vi "Progress Bar Front Panel.vi"(7 "Enable Cancel?":bool, 8 "Calling VI Ref":refnum<vi>, 9 "Main Title":string, 10 "Progress Bar Dialog":refnum<class "Loading Dialog.lvclass">, 11 "Total":i32) -> ()   [LabVIEW 2020, in "VI Properties Editor.lvlib" / "Loading Dialog.lvclass"]
doc: "The front panel for the dialog box that gets displayed."
uses:
  Loading Dialog.lvclass
  Loading Dialog.lvclass/Loading Dialog.ctl
  VI Properties Editor.lvlib
panel:
  in  "Cancelling":string="Cancelling..."
  in  "Progress Format String":string="%d of %s"
  out "Main Heading":string="Loading item data..."
  in  "Cancel":bool
  out "Status Heading":string="0 of 0"
  out "Progress Bar":dbl(slide) scale=0.0..1.0
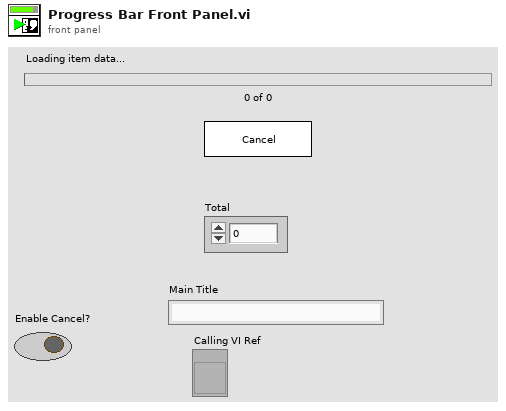
[diagram p1: front panel]
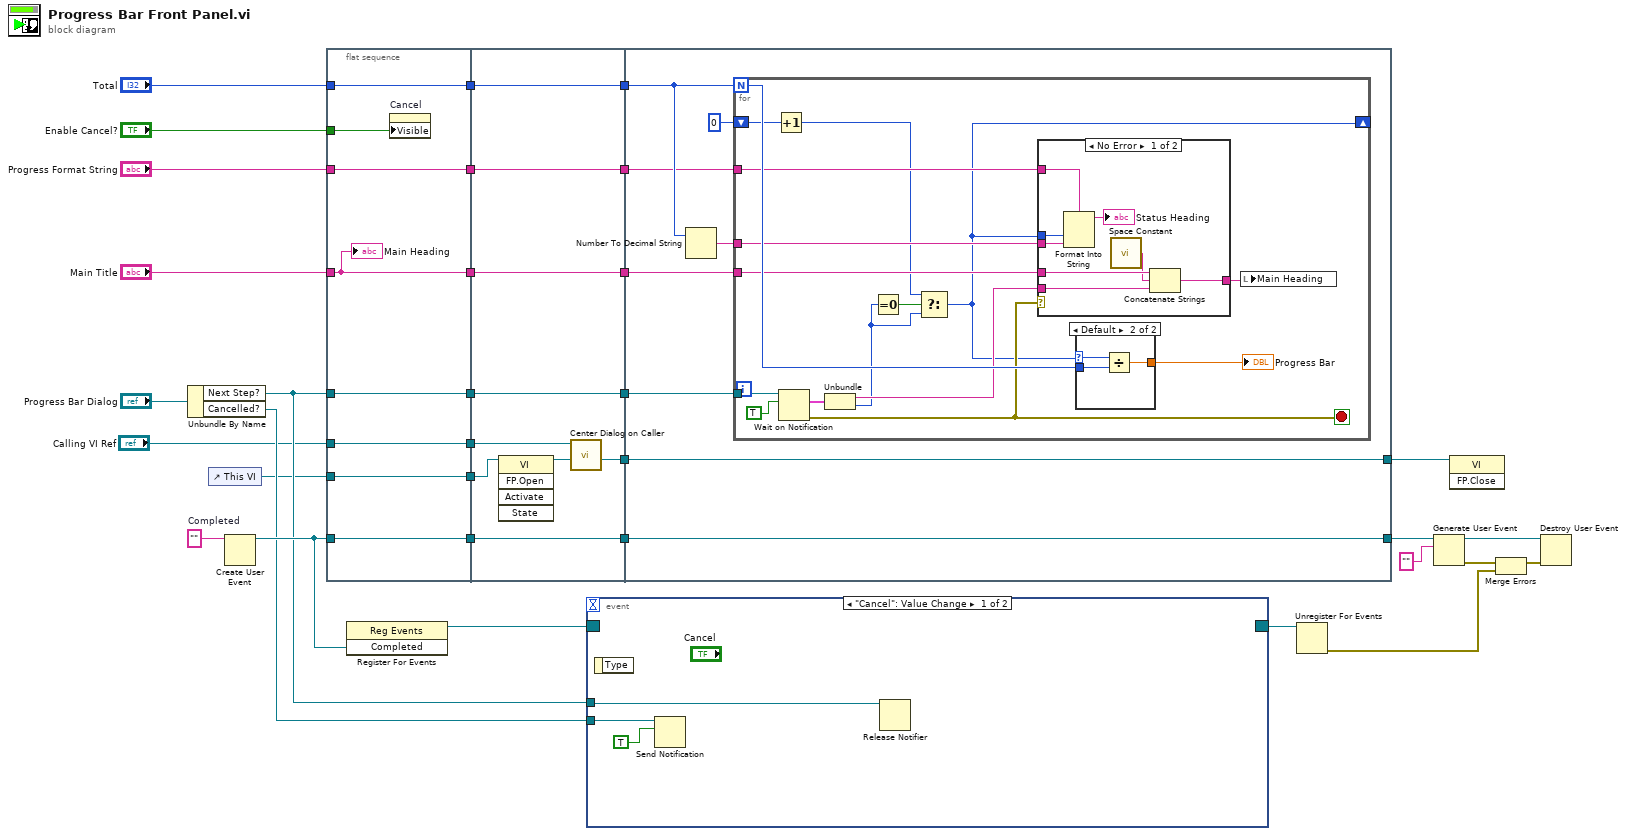
[diagram p0: block diagram]
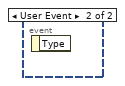
[diagram p2: hidden frame]
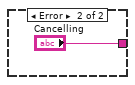
[diagram p3: hidden frame]
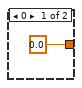
[diagram p4: hidden frame]
diagram:
  w28 = ""  # Completed
  n1 = Unbundle By Name("Progress Bar Dialog") -> ("Next Step?"=w23:refnum<notifier>, "Cancelled?"=w22:refnum<notifier>)
  n2 = control-ref of="This VI"() -> (w16:refnum<vi>)
  n3 = Create User Event(user event datatype=w28) -> (user event=w30:refnum<user-event>)  [unwired: 1 in, 1 out]
  n4 = flat-sequence {
    tunnel: [w41] -> w15
    tunnel: "Total" -> [w41]
    tunnel: "Enable Cancel?" -> [w40]
    tunnel: [w39] -> w13
    tunnel: w23 -> [w39]
    tunnel: [w38] -> w11
    tunnel: w30 -> [w38]
    tunnel: [w35] -> w9
    tunnel: [w34] -> w7
    tunnel: [w37] -> w5
    tunnel: "Calling VI Ref" -> [w37]
    tunnel: [w36] -> w4
    tunnel: w16 -> [w36]
    tunnel: "Progress Format String" -> [w35]
    tunnel: "Main Title" -> [w34]
    tunnel: w15 -> [w50]
    tunnel: [w50] -> w14
    tunnel: w13 -> [w49]
    tunnel: [w49] -> w12
    tunnel: w11 -> [w48]
    tunnel: [w48] -> w10
    tunnel: w9 -> [w47]
    tunnel: [w47] -> w8
    tunnel: w7 -> [w46]
    tunnel: [w46] -> w6
    tunnel: w5 -> [w44]
    tunnel: w4 -> [w42]
    tunnel: [w43] -> w3
    tunnel: w14 -> [w56]
    tunnel: w12 -> [w55]
    tunnel: [w54] -> w29
    tunnel: w10 -> [w54]
    tunnel: [w51] -> w21
    tunnel: w8 -> [w53]
    tunnel: w6 -> [w52]
    tunnel: w3 -> [w51]
    frame #0 {
      n5 = property on="Cancel" class="Bool"("Visible"=w40) -> ()  [unwired: 2 in, 2 out]
      "Main Heading" <- w34
    }
    frame #1 {
      n6 = invoke class="VI" method="FP.Open"(reference=w42) -> (reference out=w45:refnum<vi>)  [unwired: 4 in, 4 out]
      n7 = call "Center Dialog on Caller.vi"("Dialog VI"=w45, "Calling VI in"=w44) -> ("Dialog VI out"=w43:refnum<vi>)  [unwired: 8 in, 1 out]
    }
    frame #2 {
      n8 = Number To Decimal String(number=w56) -> (decimal integer string=w57:string)  [unwired: 1 in]
      n9 = for {
        N: w56 -> [w74]
        shift-right: [w59] -> _
        shift-left: 0 -> [w69]
        tunnel: w55 -> [w72]
        tunnel: w57 -> [w71]
        tunnel: w53 -> [w68]
        tunnel: w52 -> [w67]
        stop <- w65 stop-if-true
        n10 = Increment(x=w69) -> (x+1=w60:i32)
        n11 = Wait on Notification(notifier=w72, ignore previous (F)=TRUE) -> (notification=w64:cluster{"Name":string, "Number":i32}, error out=w65:errorcluster)  [unwired: 2 in, 2 out]
        n12 = Unbundle(w64) -> ("Name"=w63:string, "Number"=w61:i32)
        n13 = Equal To 0?(x=w61) -> (x = 0?=w62:bool)
        n14 = Select(t=w60, s=w62, f=w61) -> (s? t:f=w59:i32)
        n15 = case shown="No Error" w65 {
          tunnel: w71 -> [w82 _]
          tunnel: w59 -> [w81 _]
          tunnel: w68 -> [w80 _]
          tunnel: w67 -> [w79 _]
          tunnel: [w78 "Cancelling"] -> w66
          tunnel: w63 -> [w76 _]
          frame No Error {
            n16 = Format Into String(format string=w80, w81, w82) -> (resulting string=→"Status Heading":string)  [unwired: 2 in, 1 out]
            n17 = call <vilib>:"Space Constant.vi"() -> ("String"=w75:string)
            n18 = Concatenate Strings(w79, w75, w76) -> (w78:string)
          }
          frame Error {
          }
        }
        n19 = case shown="Default" w59 {
          selector: w59 -> [_ w87]
          tunnel: w74 -> [_ w86]
          tunnel: [0.0 w85] -> w73
          frame 0 {
          }
          frame Default {
            n20 = Divide(x=w87, y=w86) -> (x/y=w85:dbl)
          }
        }
        "Progress Bar" <- w73
        n21 = local write "Main Heading"(w66) -> ()
      }
    }
  }
  n22 = register-events(w30) -> (reference out=w31:refnum<event-registration>)  [unwired: 2 in, 1 out]
  n23 = event shown="[0] \"Cancel\": Value Change" {
    selector: w31 -> [_ _]
    dyn-events: [_ _] -> w20
    timeout: _ -> [_ _]
    tunnel: w23 -> [w90 _]
    tunnel: w22 -> [w88 _]
    event "Cancel": Value Change {
      n24 = event-data() -> ()  [unwired: 1 in, 1 out]
      n25 = Send Notification(notification=TRUE, notifier=w88) -> ()  [unwired: 1 in, 2 out]
      n26 = Release Notifier(notifier=w90) -> ()  [unwired: 2 in, 3 out]
    }
    event User Event {
      n27 = event-data() -> ()  [unwired: 1 in, 1 out]
    }
  }
  n28 = Unregister For Events(event registration refnum=w20) -> (error out=w19:errorcluster)  [unwired: 1 in]
  n29 = Generate User Event(user event=w29, event data cluster="" ("event data")) -> (user event out=w26:refnum<user-event>, error out=w27:errorcluster)  [unwired: 2 in]
  n30 = invoke class="VI" method="FP.Close"(reference=w21) -> ()  [unwired: 2 in, 3 out]
  n31 = Merge Errors(w27, w19) -> (w25:errorcluster)
  n32 = Destroy User Event(user event=w26, error in=w25) -> ()  [unwired: 1 out]
